vi "Class Implements Method.vi"(8 "error in (no error)":errorcluster, 10 "Method Name":string, 11 "Class Refnum":refnum<vi>) -> (0 "error out":errorcluster, 1 "VI Qualified Name":string, 2 "Implements method?":bool, 3 "Class Refnum out":refnum<vi>)   [LabVIEW 2020, in "Peek Window.lvlib" / "Dynamic Dispatch VI Type.lvclass"]
uses:
  Dynamic Dispatch VI Type.lvclass
  Dynamic Dispatch VI Type.lvclass/Dynamic Dispatch VI Type.ctl
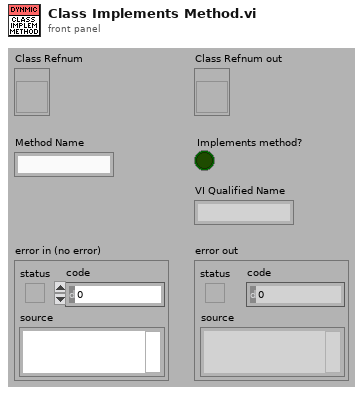
[diagram p1: front panel]
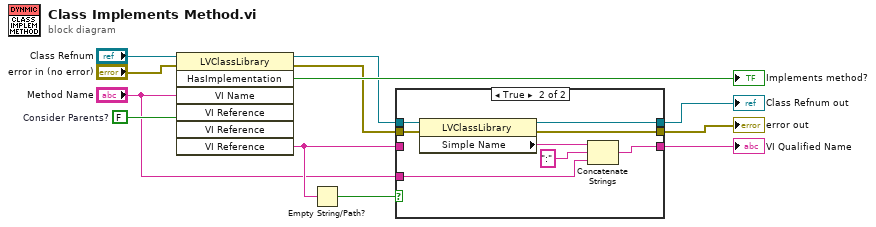
[diagram p0: block diagram]
diagram:
  w9 = FALSE  # Consider Parents?
  n1 = invoke class="LVClassLibrary" method="HasImplementation"(reference="Class Refnum", error in="error in (no error)", "VI Name"="Method Name", "VI Reference"=w9) -> (reference out=w5:refnum<vi>, error out=w6:errorcluster, "HasImplementation"=→"Implements method?":bool, "VI Reference"=w7:string)  [unwired: 3 in, 3 out]
  n2 = Empty String/Path?(string/path=w7) -> (empty?=w8:bool)
  n3 = case shown="True" w8 {
    tunnel: w7 -> [w15 _]
    tunnel: w6 -> [w13 w23]
    tunnel: w5 -> [w14 w22]
    tunnel: "Method Name" -> [_ w20]
    tunnel: [w15 w18] -> w3
    tunnel: [w14 w17] -> w1
    tunnel: [w13 w16] -> w2
    frame False {
    }
    frame True {
      n4 = property class="LVClassLibrary"(reference=w22, error in=w23) -> (reference out=w17:refnum<vi>, error out=w16:errorcluster, "Simple Name"=w21:string)
      n5 = Concatenate Strings(w21, ":", w20) -> (w18:string)
    }
  }
  "error out" <- w2
  "Class Refnum out" <- w1
  "VI Qualified Name" <- w3
